vi "Headlines.vi"() -> ()   [LabVIEW 2026]
panel:
  in  "Stop":bool
  in  "Next":bool
  in  "Mode":enum16{"Automatic", "Manual"}(ring)
  out "Current Headline":string
  out "Headline Number":dbl
  out "Total Headlines":dbl
  in  "Headlines":string[](array[string])
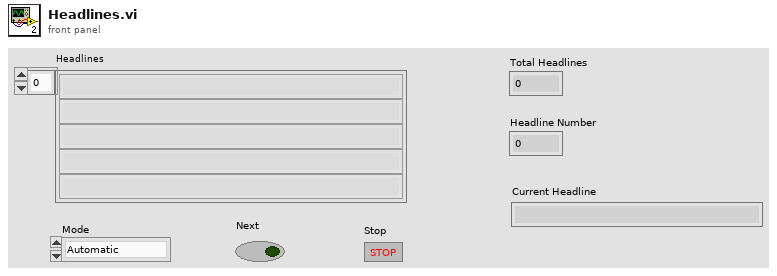
[diagram p1: front panel]
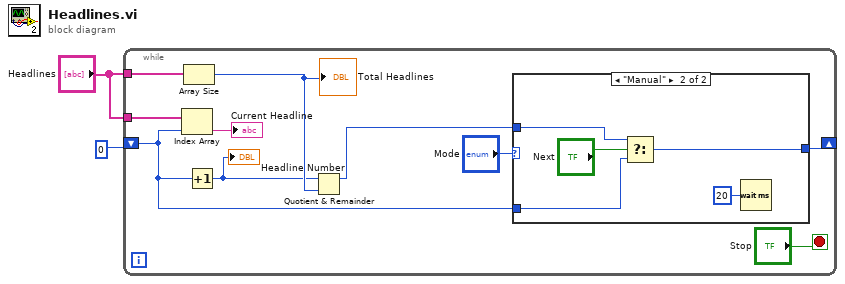
[diagram p0: block diagram]
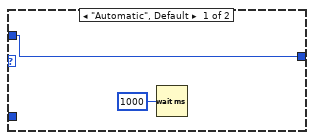
[diagram p2: hidden frame]
diagram:
  n1 = while {
    tunnel: "Headlines" -> [w11]
    shift-right: [w5] -> _
    shift-left: 0 -> [w6]
    tunnel: "Headlines" -> [w10]
    stop <- "Stop" stop-if-true
    n2 = Index Array(array=w10, index=w6) -> (element=→"Current Headline":string)
    n3 = Array Size(array=w11) -> (size(s)=w8:i32)
    "Total Headlines" <- w8
    n4 = Increment(x=w6) -> (x+1=w3:i32)
    "Headline Number" <- w3
    n5 = Quotient & Remainder(x=w3, y=w8) -> (x-y*floor(x/y)=w7:i32)  [unwired: 1 out]
    n6 = case shown="\"Manual\"" "Mode" {
      tunnel: w7 -> [w14 w18]
      tunnel: w6 -> [_ w17]
      tunnel: [w14 w16] -> w5
      frame "Automatic", Default {
        n7 = Wait (ms)(milliseconds to wait=u32 1000) -> ()  [unwired: 1 out]
      }
      frame "Manual" {
        n8 = Select(t=w18, s="Next", f=w17) -> (s? t:f=w16:i32)
        n9 = Wait (ms)(milliseconds to wait=u32 20) -> ()  [unwired: 1 out]
      }
    }
  }
